vi "Set Output Folder.vi"(8 "error in":errorcluster, 10 "Output Folder":path, 11 "Runner in":refnum<class "Runner.lvclass">) -> (0 "error out":errorcluster, 3 "Runner out":refnum<class "Runner.lvclass">)   [LabVIEW 2026, in "Runner.lvlib" / "Runner.lvclass"]
doc: "Set output folder."
uses:
  Runner.lvclass
  Runner.lvclass/Runner.ctl
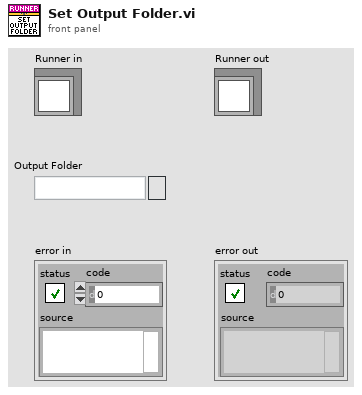
[diagram p1: front panel]
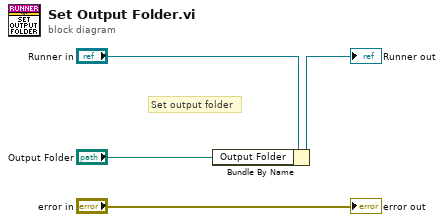
[diagram p0: block diagram]
diagram:
  # "Set output folder"
  n1 = Bundle By Name(cluster="Runner in", "Output Folder"="Output Folder") -> (→"Runner out":refnum<class "Runner.lvclass">)
  "error out" <- "error in"
